vi "laser_constant_current_output_with_DAQ_analog_output_timed_v1.vi"() -> ()   [LabVIEW 2025, in "tSNIP.lvlib"]
uses:
  tSNIP.lvlib
panel:
  in  "Current Pulse Train":T1={"Duty Cycle"={"ON"={"Units"=1, "Value"=10.0}, "OFF"={"Units"=1, "Value"=10.0}}, "Number of Cycles"=1, "Current Step"={"Value"=0.0, "Units"=0.001}, "Start Current"={"Value"=0.0, "Units"=0.001}} {"Start Current"."Units" items=["mA"=0.001, "A"=1.0]; "Current Step"."Units" items=["mA"=0.001, "A"=1.0]; "Number of Cycles" min=1; "Duty Cycle"."OFF"."Units" items=["s"=1, "min"=60, "hr"=3600]; "Duty Cycle"."ON"."Units" items=["s"=1, "min"=60, "hr"=3600]}
  out "Elapsed time":dbl format="%<%M:%S>t"
  in  "Power":cluster{"Value":dbl, "Units":dbl}={"Value"=0.0, "Units"=0.001} {"Units" items=["mW"=0.001, "W"=1.0]}
  out "Current":cluster{"Value":dbl, "Units":dbl}={"Value"=0.0, "Units"=0.001} {"Units" items=["mA"=0.001, "A"=1.0]}
  in  "DAQmx Device":tag
  in  "VISA resource name":refnum<visa-resource-name>
  in  "Laser Active":bool
  in  "EXIT":bool
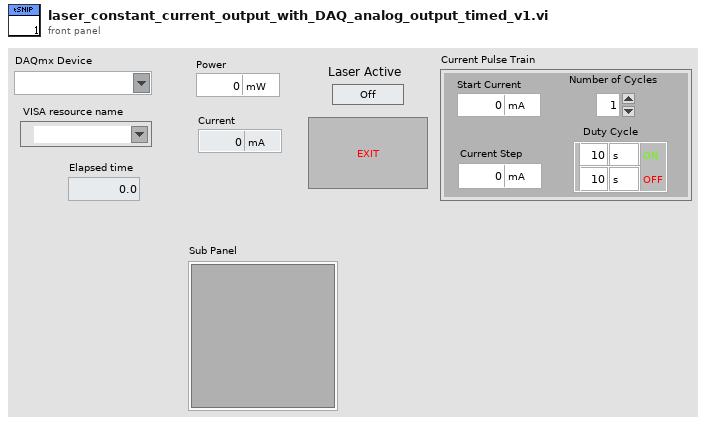
[diagram p1: front panel]
types:
  T1 = cluster{"Duty Cycle":cluster{"ON":cluster{"Units":u16, "Value":dbl}, "OFF":cluster{"Units":u16, "Value":dbl}}, "Number of Cycles":u64, "Current Step":cluster{"Value":dbl, "Units":dbl}, "Start Current":cluster{"Value":dbl, "Units":dbl}}
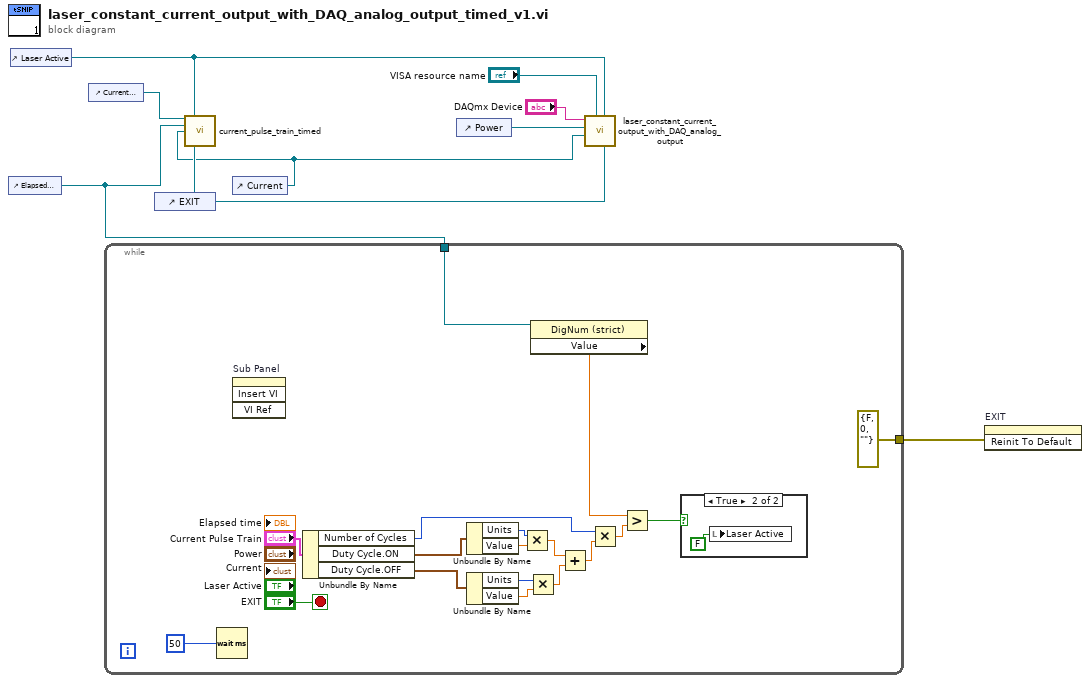
[diagram p0: block diagram]
diagram:
  n1 = control-ref of="Elapsed time"() -> (w3:refnum<vi>)
  n2 = control-ref of="Laser Active"() -> (w5:refnum<vi>)
  n3 = control-ref of="Current Pulse Train"() -> (w6:refnum<vi>)
  n4 = while {
    tunnel: [errorcluster {"status"=FALSE, "code"=0, "source"=""} ("error in (no error)")] -> w7
    tunnel: w3 -> [w20]
    stop <- "EXIT" stop-if-true
    n5 = Wait (ms)(milliseconds to wait=u32 50) -> ()  [unwired: 1 out]
    n6 = invoke on="Sub Panel" class="SubPnl" method="Insert VI"() -> ()  [unwired: 4 in, 4 out]
    n7 = Unbundle By Name("Current Pulse Train") -> ("Number of Cycles"=w10:u64, "Duty Cycle.ON"=w11:cluster{"Units":u16, "Value":dbl}, "Duty Cycle.OFF"=w16:cluster{"Units":u16, "Value":dbl})
    n8 = Unbundle By Name(w11) -> ("Units"=w24:u16, "Value"=w23:dbl)
    n9 = Unbundle By Name(w16) -> ("Units"=w18:u16, "Value"=w17:dbl)
    n10 = Multiply(x=w24, y=w23) -> (x*y=w15:dbl)
    n11 = Multiply(x=w18, y=w17) -> (x*y=w14:dbl)
    n12 = property class="DigNum (strict)"(reference=w20) -> ("Value"=w19:dbl)  [unwired: 1 in, 2 out]
    n13 = Add(x=w15, y=w14) -> (x+y=w12:dbl)
    n14 = Multiply(x=w10, y=w12) -> (x*y=w13:dbl)
    n15 = Greater?(x=w19, y=w13) -> (0:w22:bool)
    n16 = case shown="True" w22 {
      frame False {
      }
      frame True {
        n17 = local write "Laser Active"(FALSE) -> ()
      }
    }
  }
  n18 = control-ref of="EXIT"() -> (w4:refnum<vi>)
  n19 = control-ref of="Current"() -> (w1:refnum<vi>)
  n20 = call "current_pulse_train_timed.vi"("Current Train Ref"=w6, "Laser Active Ref"=w5, "Elapsed Time Ref"=w3, "Instantaneous Current Ref"=w1, "Exit Ref"=w4) -> ()  [unwired: 10 in, 1 out]
  n21 = control-ref of="Power"() -> (w2:refnum<vi>)
  n22 = call "laser_constant_current_output_with_DAQ_analog_output.vi"("Exit Refnum"=w4, "Activate Refnum"=w5, "VISA resource name"="VISA resource name", "Current Refnum"=w1, "Power Refnum"=w2, "DAQmx Device"="DAQmx Device") -> ()  [unwired: 5 in, 1 out]
  n23 = invoke on="EXIT" class="Bool (strict)" method="Reinit To Default"(error in=w7) -> ()  [unwired: 2 in, 3 out]
